vi "query HO UL_DL Center Channel Number.vi"(8 "error in (no error)":errorcluster caption="에러 입력(에러 없음)", 9 "Direction":T2, 10 "Selected CC Argements":T1, 11 "NR 입력":refnum<class "NR.lvclass">) -> (0 "error out":errorcluster caption="에러 출력", 2 "Center Channel Number":u32, 3 "NR 출력":refnum<class "NR.lvclass">)   [LabVIEW 2023, in "ANRITSU Call Box.lvlib" / "NR.lvclass"]
uses:
  NR.lvclass
  NR.lvclass/NR.ctl
  Type Definition/Uplink Downlink Enum.ctl
  ANRITSU Call Box.lvlib
  Type Definition/NR Selected CC Type Arguments.ctl
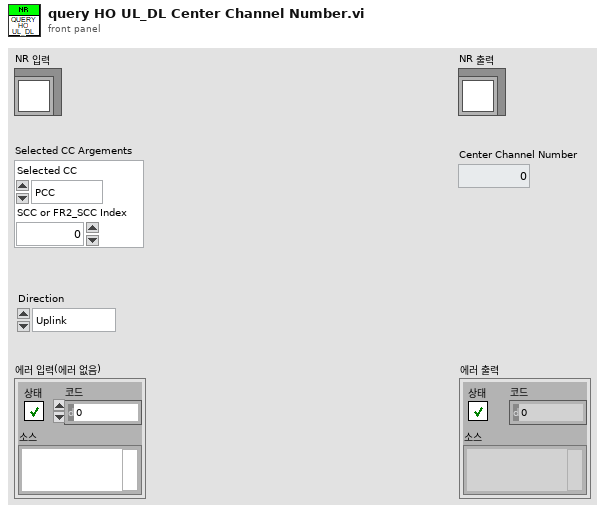
[diagram p1: front panel]
types:
  T1 = typedef "ANRITSU Call Box.lvlib/NR Selected CC Type Arguments.ctl" = cluster{"Selected CC":enum16{"PCC", "SCC", "FR2_PCC", "FR2_SCC"}, "SCC or FR2_SCC Index":u32}
  T2 = typedef "ANRITSU Call Box.lvlib/Uplink Downlink Enum.ctl" = enum16{"Uplink", "Downlink"}
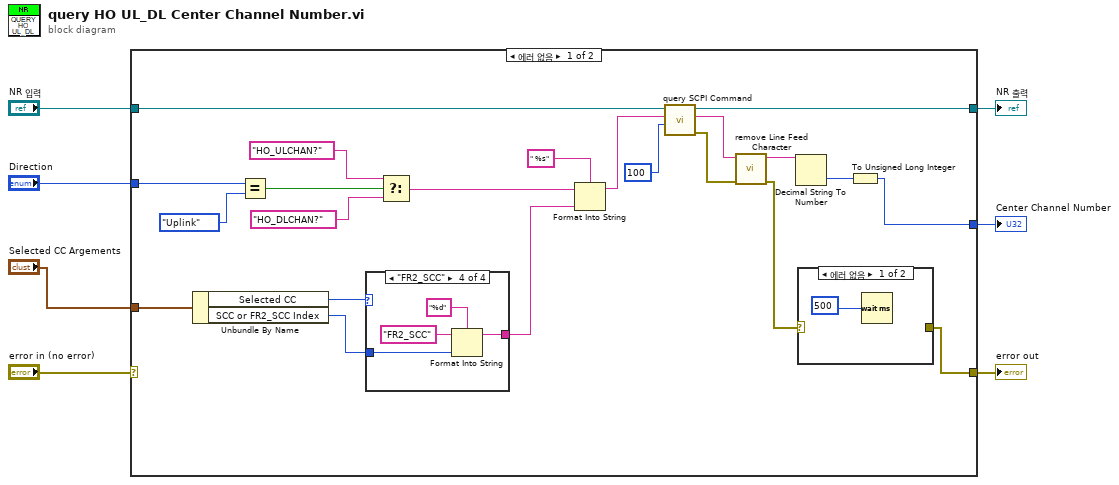
[diagram p0: block diagram]
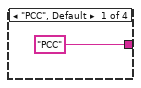
[diagram p3: hidden frame]
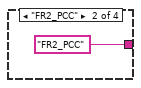
[diagram p4: hidden frame]
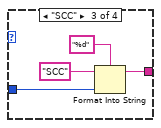
[diagram p5: hidden frame]
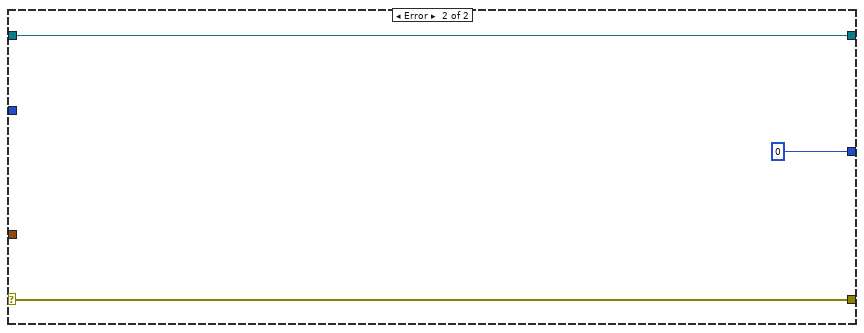
[diagram p6: hidden frame]
diagram:
  n1 = case shown="에러 없음" "error in (no error)" {
    selector: "error in (no error)" -> [_ w44]
    tunnel: [w11 w44] -> w6
    tunnel: [w13 w43] -> w4
    tunnel: "NR 입력" -> [w14 w43]
    tunnel: [w12 u32 0] -> w3
    tunnel: "Direction" -> [w10 _]
    tunnel: "Selected CC Argements" -> [w9 _]
    frame No Error {
      n2 = Unbundle By Name(w9) -> ("Selected CC"=w8:enum16{"PCC", "SCC", "FR2_PCC", "FR2_SCC"}, "SCC or FR2_SCC Index"=w21:u32)
      n3 = Equal?(x=w10, y=Uplink_Downlink_Enum."Uplink") -> (x = y?=w20:bool)
      n4 = case shown="\"FR2_SCC\"" w8 {
        tunnel: ["PCC" "FR2_PCC" w35 w39] -> w23
        tunnel: w21 -> [_ _ w34 w38]
        frame "PCC", Default {
        }
        frame "FR2_PCC" {
        }
        frame "SCC" {
          n5 = Format Into String(format string="%d", initial string="SCC", w34) -> (resulting string=w35:string)  [unwired: 1 in, 1 out]
        }
        frame "FR2_SCC" {
          n6 = Format Into String(format string="%d", initial string="FR2_SCC", w38) -> (resulting string=w39:string)  [unwired: 1 in, 1 out]
        }
      }
      n7 = Select(t="HO_ULCHAN?", s=w20, f="HO_DLCHAN?") -> (s? t:f=w22:string)
      n8 = Format Into String(format string=" %s", initial string=w22, w23) -> (resulting string=w24:string)  [unwired: 1 in, 1 out]
      n9 = call "query SCPI Command.vi"("Read Buffer Length"=u32 100, "SCPI Command"=w24, "NR in"=w14) -> ("error out"=w26:errorcluster, "Read Buffer String"=w25:string, "NR out"=w13:refnum<class "NR.lvclass">)  [unwired: 6 in]
      n10 = call "remove Line Feed Character.vi"("error in"=w26, "Query String"=w25) -> ("error out"=w29:errorcluster, "Line Feed Removed String"=w28:string)  [unwired: 8 in]
      n11 = Decimal String To Number(string=w28) -> (number=w27:i32)  [unwired: 2 in, 1 out]
      n12 = case shown="에러 없음" w29 {
        selector: w29 -> [_ w31]
        tunnel: [_ w31] -> w11
        frame No Error {
          n13 = Wait (ms)(milliseconds to wait=u32 500) -> ()  [unwired: 1 out]
        }
        frame Error {
        }
      }
      n14 = To Unsigned Long Integer(number=w27) -> (unsigned 32bit integer=w12:u32)
    }
    frame Error {
    }
  }
  "error out" <- w6
  "NR 출력" <- w4
  "Center Channel Number" <- w3
